vi "UI Servo Parameters Monitor .vi"() -> ()   [LabVIEW 2021]
uses:
  <vilib>/Utility/miscctls.llb/LVRowAndColumnTypeDef.ctl
  <vilib>/Utility/file.llb/Read Delimited Spreadsheet (string).vi
  <vilib>/NI/Modbus Library/API/Wrapper/Create TCP Slave.vi
  <vilib>/NI/Modbus Library/API/Slave/Modbus Slave.lvclass
  <vilib>/NI/Modbus Library/API/Wrapper/API Main.lvlib
panel:
  in  "Tab Control":enum32{"Page 1", "Page 2"}(tab)
  in  "Button 2":bool
  in  "Button":bool
  in  "New Value":dbl
  out "Servo Parameter List":string[][](table)
  in  "stop modbus loop":bool
  out "Active Cell:Active Cell":T1
  in  "Parameters:":i32(listbox)
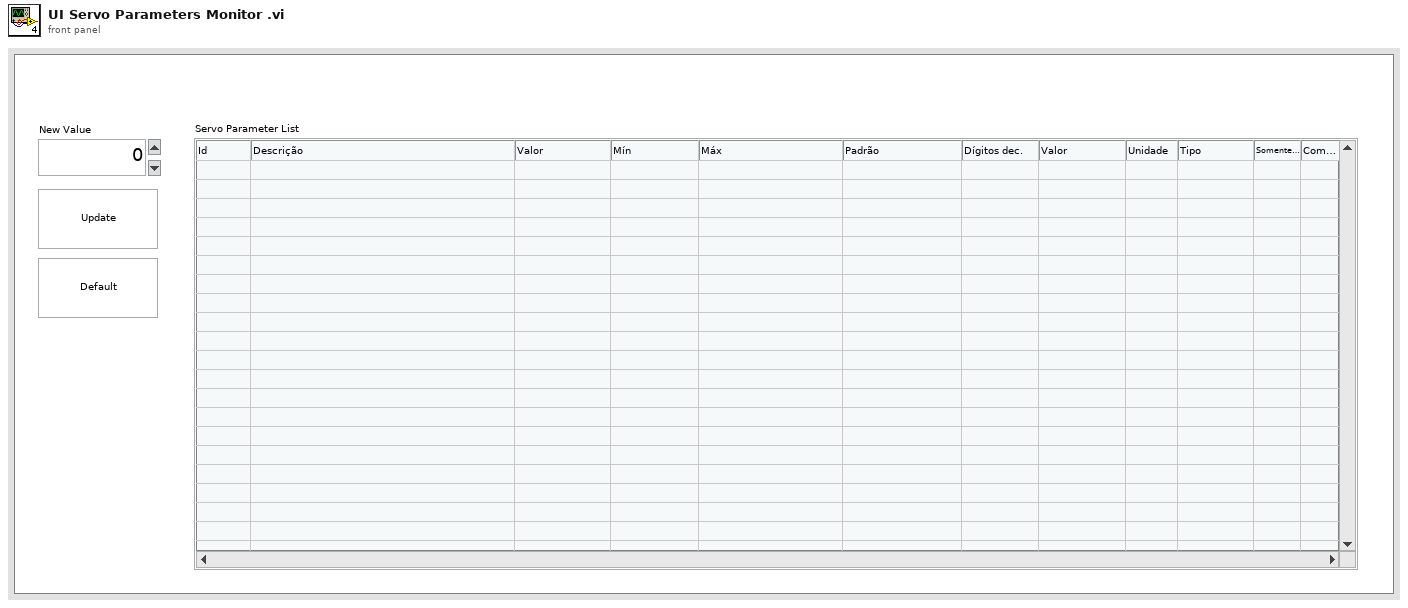
[diagram p1: front panel]
types:
  T1 = typedef "LVRowAndColumnTypeDef.ctl" = cluster{"Row":i32, "Column":i32}
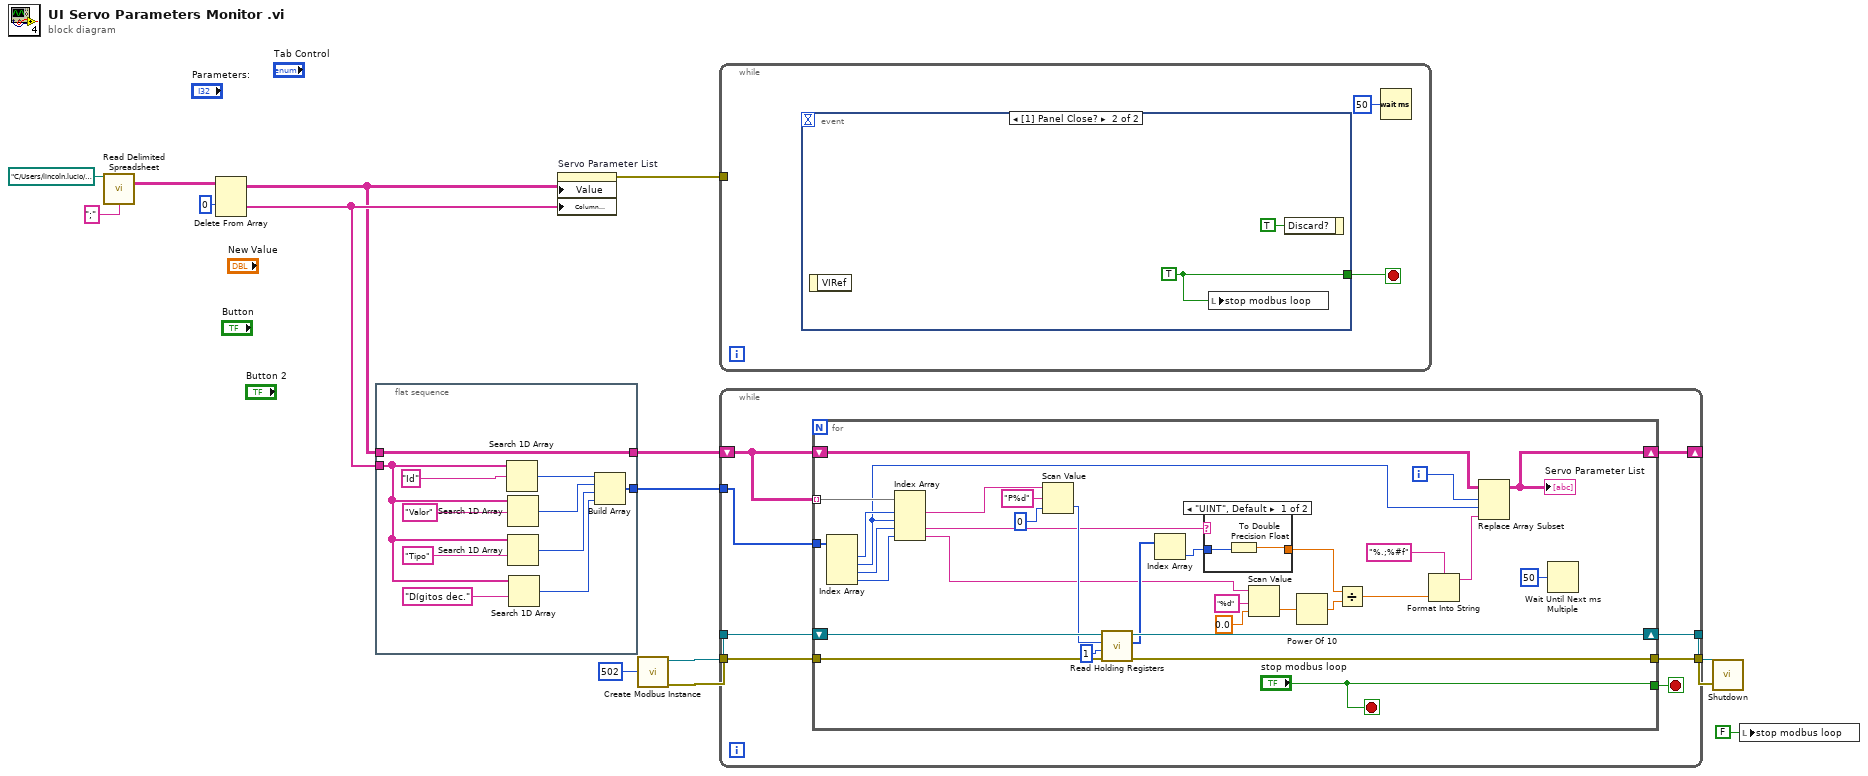
[diagram p0: block diagram]
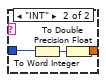
[diagram p2: hidden frame]
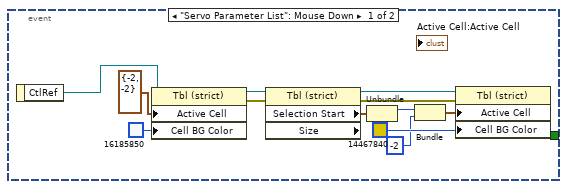
[diagram p3: hidden frame]
diagram:
  n1 = call-poly <vilib>:"Read Delimited Spreadsheet.vi"("file path (dialog if empty)"=path "C:/Users/lincoln.lucio/Documents/Lincoln/Documentos Pessoais/meus docs/Projetos pessoais/Projeto Sciranda/sciranda/documentos/parameters list.csv", "delimiter (\\t)"=";" ("delimiter (\\t)")) -> ("all rows"=w2:string[][])  [unwired: 8 in, 5 out]
  n2 = Delete From Array(array=w2, index (row)=0 ("index")) -> (deleted portion=w6:string[], array with subset deleted=w1:string[][])  [unwired: 2 in]
  n3 = flat-sequence {
    tunnel: [w18] -> w7
    tunnel: w6 -> [w16]
    tunnel: w1 -> [w17]
    tunnel: [w17] -> w5
    frame #0 {
      n4 = Search 1D Array(1D array=w16, element="Id") -> (index of element=w22:i32)  [unwired: 1 in]
      n5 = Search 1D Array(1D array=w16, element="Valor") -> (index of element=w21:i32)  [unwired: 1 in]
      n6 = Search 1D Array(1D array=w16, element="Tipo") -> (index of element=w20:i32)  [unwired: 1 in]
      n7 = Search 1D Array(1D array=w16, element="Dígitos dec.") -> (index of element=w19:i32)  [unwired: 1 in]
      n8 = Build Array(w22, w21, w20, w19) -> (w18:i32[])
    }
  }
  n9 = property on="Servo Parameter List" class="Tbl (strict)"("Value"=w1, "Column Headers[]"=w6) -> (error out=w12:errorcluster)  [unwired: 2 in, 1 out]
  n10 = call-poly <vilib>:"Create Modbus Instance.vi"("port (502)"=u16 502) -> ("error out"=w10:errorcluster, "TCP slave instance"=w11:refnum<class "Modbus Slave.lvclass">)  [unwired: 9 in]
  n11 = while {
    tunnel: w12 -> [_]
    stop <- w27 stop-if-true
    n12 = event shown="[1] Panel Close?" {
      selector: _ -> [_ _]
      dyn-events: _ -> [_ _]
      timeout: _ -> [_ _]
      tunnel: [_ w41] -> w27
      event "Servo Parameter List": Mouse Down {
        n13 = event-data() -> ("CtlRef"=w33:refnum<vi>)  [unwired: 1 in]
        n14 = property class="Tbl (strict)"(reference=w33, "Active Cell"=T1 {"Row"=-2, "Column"=-2} ("Selection Start"), "Cell BG Color"=u32 16185850 ("Active Cell:Cell Background Color")) -> (reference out=w34:refnum<vi>, error out=w35:errorcluster)  [unwired: 1 in]
        n15 = property class="Tbl (strict)" props=["Selection Start", "Size"](reference=w34, error in=w35) -> (reference out=w40:refnum<vi>, error out=w39:errorcluster, "Selection Start"=w32:T1)  [unwired: 1 out]
        n16 = Unbundle(w32) -> ("Row"=w31:i32)  [unwired: 1 out]
        n17 = Bundle("Row"=w31, "Column"=-2) -> (w30:cluster{"Row":i32, "Column":i32})  [unwired: 1 in]
        n18 = property class="Tbl (strict)"(reference=w40, error in=w39, "Active Cell"=w30, "Cell BG Color"=u32 14467840 ("Active Cell:Cell Background Color")) -> ()  [unwired: 2 out]
      }
      event Panel Close? {
        w41 = TRUE
        n19 = event-data() -> ()  [unwired: 1 in, 1 out]
        n20 = local write "stop modbus loop"(w41) -> ()
        n21 = event-data("Discard?"=TRUE) -> ()  [unwired: 1 in, 1 out]
      }
    }
    n22 = Wait (ms)(milliseconds to wait=u32 50) -> ()  [unwired: 1 out]
  }
  n23 = while {
    tunnel: w11 -> [w50]
    tunnel: w10 -> [w49]
    tunnel: [w48] -> w9
    tunnel: [w47] -> w8
    tunnel: w7 -> [w46]
    shift-right: [w43] -> _
    shift-left: w5 -> [w44]
    stop <- w45 stop-if-true
    n24 = for {
      shift-right: [w80] -> w48
      shift-left: w50 -> [w82]
      tunnel: w49 -> [w81]
      tunnel: [w79] -> w47
      tunnel: w44 -> [w75] mode=indexing
      tunnel: w46 -> [w74]
      tunnel: ["stop modbus loop"] -> w45
      shift-right: [w52] -> w43
      shift-left: w44 -> [w54]
      i -> [w55]
      stop <- "stop modbus loop" stop-if-true
      n25 = Index Array(array=w74) -> (element #1=w78:i32, element #2=w51:i32, element #3=w77:i32, element #4=w76:i32)  [unwired: 4 in]
      n26 = Index Array(array=w75, index #1=w78, index #2=w51, index #3=w77, index #4=w76) -> (element #1=w71:string, element #3=w68:string, element #4=w62:string)  [unwired: 1 out]
      n27 = Scan Value(string=w71, format string="P%d", default (0 dbl)=u16 0 ("default value 1")) -> (value=w70:u16)  [unwired: 1 out]
      n28 = call-dynamic "Read Holding Registers.vi"("error in"=w81, "number of inputs"=u16 1, "starting address"=w70, "Modbus slave in"=w82) -> ("error out"=w79:errorcluster, "register values"=w67:u16[], "Modbus slave out"=w80:refnum<class "Modbus Slave.lvclass">)  [unwired: 5 in]
      n29 = Index Array(array=w67) -> (element=w66:u16)  [unwired: 1 in]
      n30 = case shown="\"UINT\", Default" w68 {
        tunnel: w66 -> [w84 w87]
        tunnel: [w83 w85] -> w60
        frame "UINT", Default {
          n31 = To Double Precision Float(number=w84) -> (double precision float=w83:dbl)
        }
        frame "INT" {
          n32 = To Word Integer(number=w87) -> (16bit integer=w86:i16)
          n33 = To Double Precision Float(number=w86) -> (double precision float=w85:dbl)
        }
      }
      n34 = Scan Value(string=w62, format string="%d", default (0 dbl)=0.0 ("default value 1")) -> (value=w63:dbl)  [unwired: 1 out]
      n35 = Power Of 10(x=w63) -> (10^x=w61:dbl)
      n36 = Divide(x=w60, y=w61) -> (x/y=w57:dbl)
      n37 = Format Into String(format string="%.;%#f", w57) -> (resulting string=w56:string)  [unwired: 2 in, 1 out]
      n38 = Replace Array Subset(array=w54, new element=w56, index (row)=w55, index (col)=w51) -> (w52:string[][])
      "Servo Parameter List" <- w52
      n39 = Wait Until Next ms Multiple(millisecond multiple=u32 50 ("milliseconds to wait")) -> ()  [unwired: 1 out]
    }
  }
  n40 = call-dynamic "Shutdown.vi"("error in"=w8, "Modbus slave in"=w9) -> ()  [unwired: 9 in, 1 out]
  n41 = local write "stop modbus loop"(FALSE ("stop modbus loop")) -> ()
